vi "Plot Time Range.vi"(6 "Swap Axes":bool, 8 "End":dbl format="%<%H:%M:%S%1u>T", 9 "Start":dbl format="%<%H:%M:%S%1u>T", 11 "Plot Data":cluster{"X":dbl[], "Y":dbl[]}) -> (0 "Actual End":dbl format="%<%H:%M:%S%1u>T", 1 "Actual Start":dbl format="%<%H:%M:%S%1u>T", 2 "Independent":dbl[](array[numeric]), 3 "Dependent":dbl[](array[numeric]))   [LabVIEW 2020, in "VolatusGUIElements.lvlib"]
uses:
  VolatusGUIElements.lvlib
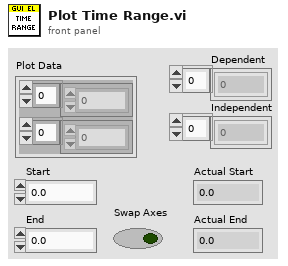
[diagram p1: front panel]
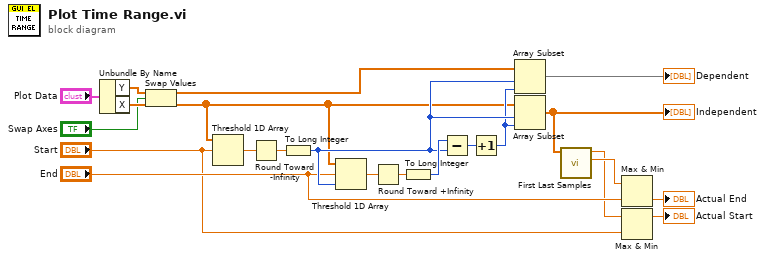
[diagram p0: block diagram]
diagram:
  n1 = Unbundle By Name("Plot Data") -> ("Y"=w5:dbl[], "X"=w4:dbl[])
  n2 = Swap Values(12:w5, 13:"Swap Axes", 14:w4) -> (1:w1:dbl[], 3:w2:dbl[])
  n3 = Threshold 1D Array(2:"Start", 3:w2) -> (0:w21:dbl)  [unwired: 1 in]
  n4 = Round Toward -Infinity(1:w21) -> (0:w20:dbl)
  n5 = To Long Integer(number=w20) -> (32bit integer=w15:i32)
  n6 = Threshold 1D Array(1:w15, 2:"End", 3:w2) -> (0:w19:dbl)
  n7 = Round Toward +Infinity(x=w19) -> (ceil(x): smallest int >= x=w18:dbl)
  n8 = To Long Integer(number=w18) -> (32bit integer=w17:i32)
  n9 = Subtract(x=w17, y=w15) -> (x-y=w16:i32)
  n10 = Increment(x=w16) -> (x+1=w14:i32)
  n11 = Array Subset(array=w1, index=w15, length=w14) -> (→"Dependent":dbl[])
  n12 = Array Subset(array=w2, index=w15, length=w14) -> (w12:dbl[])
  "Independent" <- w12
  n13 = call "First Last Samples.vi"("Data"=w12) -> ("Last"=w11:dbl, "First"=w8:dbl)  [unwired: 9 in]
  n14 = Max & Min(x=w11, y="End") -> (min(x,y)=→"Actual End":dbl)  [unwired: 1 out]
  n15 = Max & Min(x=w8, y="Start") -> (max(x,y)=→"Actual Start":dbl)  [unwired: 1 out]
